vi "RemoteVI JSON String.vi"(0 "text":u16[](array[numeric])) -> (4 "json":string)   [LabVIEW 2020, in "RemoteVI.lvlib"]
doc: "Turns UTF-16 text (code units, e.g. a window caption from user32 GetWindowTextW.vi) into a JSON string literal made of ASCII only, quotes included: printable ASCII 0x20-0x7E is kept as it is except \" and \\, every other code unit is written as \\u followed by four hex digits (LabVIEW writes them upper case) (a surrogate pair as two such escapes, which JSON allows). So any caption travels in a WebSocket text message, which must be valid UTF-8, whatever the host's code page - LabVIEW strings are bytes in the system code page, and a caption narrowed to them would be neither UTF-8 nor reversible. Pure function, cannot fail. Used for the windows message (docs\\protocol.md section 7)."
uses:
  RemoteVI.lvlib
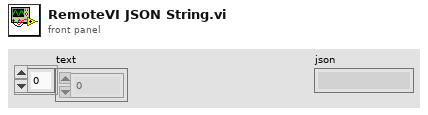
[diagram p1: front panel]
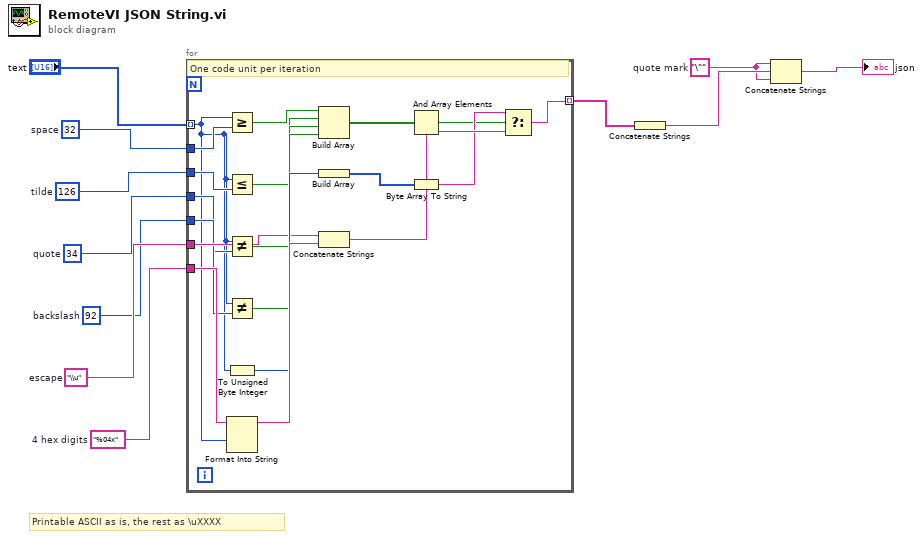
[diagram p0: block diagram]
diagram:
  w9 = "\""  # quote mark
  w7 = "%04x"  # 4 hex digits
  w6 = "\\u"  # escape
  w5 = u16 92  # backslash
  w4 = u16 34  # quote
  w3 = u16 126  # tilde
  w2 = u16 32  # space
  # "Printable ASCII as is, the rest as \\uXXXX"
  n1 = for {
    tunnel: "text" -> [w12] mode=indexing
    tunnel: w2 -> [w13]
    tunnel: w3 -> [w14]
    tunnel: w4 -> [w15]
    tunnel: w5 -> [w16]
    tunnel: w6 -> [w17]
    tunnel: w7 -> [w18]
    tunnel: [w30] -> w8 mode=indexing
    # "One code unit per iteration"
    n2 = Greater Or Equal?(x=w12, y=w13) -> (x >= y?=w19:bool)
    n3 = Less Or Equal?(x=w12, y=w14) -> (x <= y?=w20:bool)
    n4 = Not Equal?(x=w12, y=w15) -> (x != y?=w21:bool)
    n5 = Not Equal?(x=w12, y=w16) -> (x != y?=w22:bool)
    n6 = To Unsigned Byte Integer(number=w12) -> (unsigned 8bit integer=w25:u8)
    n7 = Format Into String(format string=w18, w12) -> (resulting string=w28:string)  [unwired: 2 in, 1 out]
    n8 = Build Array(w19, w20, w21, w22) -> (w23:bool[])
    n9 = Build Array(w25) -> (w26:u8[])
    n10 = Concatenate Strings(w17, w28) -> (w29:string)
    n11 = And Array Elements(Boolean array=w23) -> (logical AND=w24:bool)
    n12 = Byte Array To String(unsigned byte array=w26) -> (string=w27:string)
    n13 = Select(t=w27, s=w24, f=w29) -> (s? t:f=w30:string)
  }
  n14 = Concatenate Strings(w8) -> (w10:string)
  n15 = Concatenate Strings(w9, w10, w9) -> (→"json":string)
